vi "Startup.vi"(7 "IP Address (localhost)":string, 8 "error in (no error)":errorcluster, 9 "max connections (0: no limit)":u32, 10 "TCP port (50007)":u16=50007) -> (0 "error out":errorcluster, 3 "JKI_Python_Server out":refnum<class "Server.lvclass">)   [LabVIEW 2020, in "jki_python_bridge.lvlib" / "Server.lvclass"]
uses:
  Server.lvclass
  Server.lvclass/Server.ctl
  Type Definitions/Class Private Data - Cluster.ctl
  Type Definitions/Public Events - Cluster.ctl
  Type Definitions/Python Node.ctl
  PyObject/PyObject.lvclass
  Call/Call.lvclass
  Support/Python TCP Connection Handler.vi
  <vilib>/addons/_JKI.lib/_JKI_lib_TCP_Server.llb/JKI TCP Server.lvclass
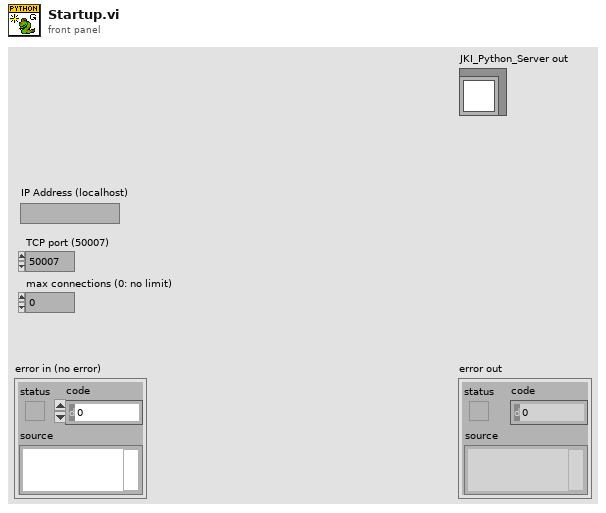
[diagram p1: front panel]
types:
  T1 = typedef "jki_python_bridge.lvlib/Server.lvclass/Class Private Data - Cluster.ctl" = cluster{"TCP Server Refnum":refnum<class "JKI TCP Server.lvclass">, "TCP port (50007)":u16, "max connections (0: no limit)":u32, "net address (0: Listen on All Adaptors)":u32, "Nodes":T2[], "Public Events":T3}
  T2 = typedef "jki_python_bridge.lvlib/Server.lvclass/Python Node.ctl" = cluster{"Name":string, "Python Method Call":refnum<user-event>, "Call Handle":refnum<class "PyObject.lvclass">}
  T3 = typedef "jki_python_bridge.lvlib/Server.lvclass/Public Events - Cluster.ctl" = cluster{"Stop Nodes":refnum<user-event>}
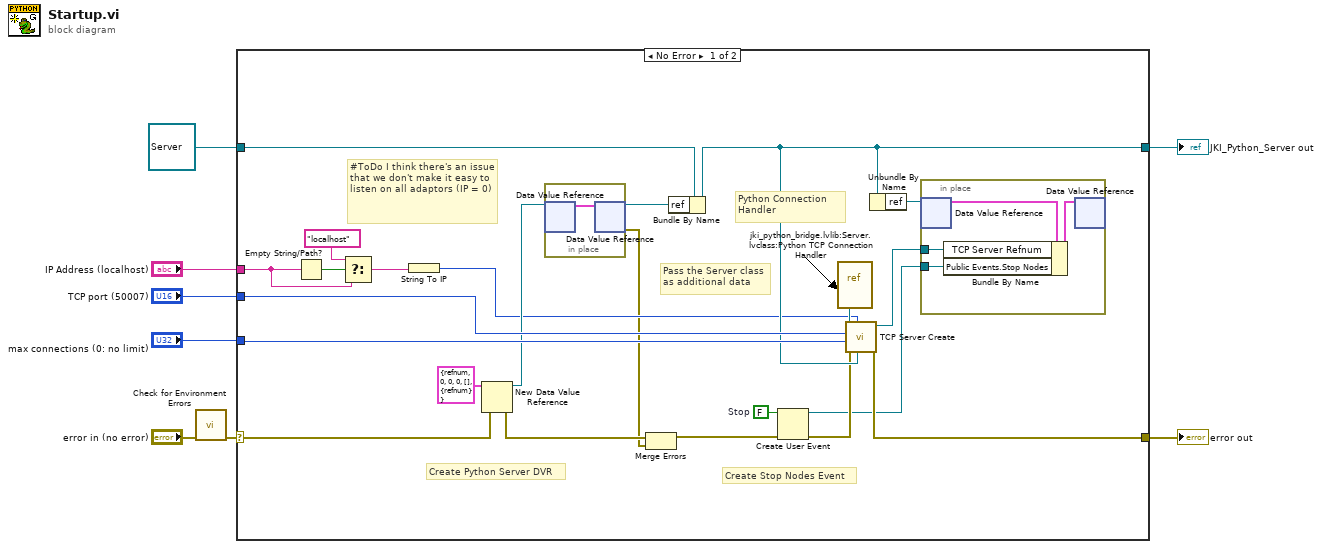
[diagram p0: block diagram]
diagram:
  n1 = call "Check for Environment Errors.vi"("error in (no error)"="error in (no error)") -> ("error out"=w1:errorcluster)  [unwired: 10 in]
  n2 = case shown="No Error" w1 {
    selector: w1 -> [w25 w38]
    tunnel: [w28 w38] -> w8
    tunnel: [w27 w37] -> w6
    tunnel: refnum<class "Server.lvclass"> refnum ("JKI_Python_Server in") -> [w31 w37]
    tunnel: "TCP port (50007)" -> [w29 _]
    tunnel: "max connections (0: no limit)" -> [w30 _]
    tunnel: "IP Address (localhost)" -> [w26 _]
    frame No Error {
      w13 = FALSE  # Stop
      # "#ToDo I think there's an issue that we don't make it easy to listen on all adaptors (IP = 0)"
      # "Create Stop Nodes Event"
      # "Create Python Server DVR"
      # "Pass the Server class\nas additional data"
      # "Python Connection \nHandler"
      n3 = Empty String/Path?(string/path=w26) -> (empty?=w11:bool)
      n4 = Select(t="localhost" ("f"), s=w11, f=w26) -> (s? t:f=w16:string)
      n5 = String To IP(1:w16) -> (0:w18:u32)
      n6 = New Data Value Reference(data value=T1 {"TCP Server Refnum"=refnum, "TCP port (50007)"=0, "max connections (0: no limit)"=0, "net address (0: Listen on All Adaptors)"=0, "Nodes"=[], "Public Events"={"Stop Nodes"=refnum}} ("Private Data"), error in=w25) -> (data value reference=w23:refnum<data-value>, error out=w10:errorcluster)
      n7 = in-place {
        n8 = in-place-dvr #1(w23) -> (w36:T1)  [unwired: 1 out]
        n9 = in-place-dvr #1(w36) -> (w22:refnum<data-value>, w9:errorcluster)
      }
      n10 = Merge Errors(w10, w9) -> (w15:errorcluster)
      n11 = Bundle By Name(cluster=w31, "ref"=w22) -> (w27:refnum<class "Server.lvclass">)
      n12 = Create User Event(user event datatype=w13, error in=w15) -> (user event=w12:refnum<user-event>, error out=w14:errorcluster)
      n13 = vi-ref "jki_python_bridge.lvlib:Server.lvclass:Python TCP Connection Handler.vi"() -> ("vi reference"=w21:refnum<vi>)
      n14 = call <vilib>:"TCP Server Create.vi"("Additional Data"=w27, "net address (0: Listen on All Adaptors)"=w18, "error in (no error)"=w14, "max connections (0: no limit)"=w30, "port"=w29, "Connection Handler Call-Back VI RefNum"=w21) -> ("error out"=w28:errorcluster, "TCP Server"=w20:refnum<class "JKI TCP Server.lvclass">)  [unwired: 4 in]
      n15 = Unbundle By Name(w27) -> ("ref"=w19:refnum<data-value>)
      n16 = in-place {
        in-place-border: w20 -> [w35]
        in-place-border: w12 -> [w32]
        n17 = in-place-dvr #2(w19) -> (w34:T1)  [unwired: 1 out]
        n18 = Bundle By Name(cluster=w34, "TCP Server Refnum"=w35, "Public Events.Stop Nodes"=w32) -> (w33:T1)
        n19 = in-place-dvr #2(w33) -> ()  [unwired: 2 out]
      }
    }
    frame Error {
    }
  }
  "error out" <- w8
  "JKI_Python_Server out" <- w6
